vi "Refresh Scalar Channels.vi"(6 "scalar channels":T1[](array[typedef]) {"Data Type" format="%.0x"}, 8 "error in (no error)":errorcluster, 9 "scalar type GUID":string, 11 "scalar section ref in":T3 format="%.0x") -> (0 "error out":errorcluster, 3 "scalar section ref out":T3 format="%.0x")   [LabVIEW 2020, in "FPGA Addon System Explorer.lvlib"]
uses:
  FPGA Addon System Explorer.lvlib
  <vilib>/NI VeriStand/Custom Device API/Custom Device Item Ref.ctl
  Addon Shared/Types/Register Information.ctl
  Addon Shared/Types/FPGA Addon Data Type.ctl
  <vilib>/NI VeriStand/Custom Device Tools/Custom Device Utility Library/NI VeriStand - Search for Item by GUID.vi
  <vilib>/NI VeriStand/Custom Device Tools/Custom Device Utility Library/Custom Device Utility Library.lvlib
  <vilib>/NI VeriStand/Custom Device API/Custom Device API.lvlib
  Addon Shared/FPGA Addon Shared.lvlib
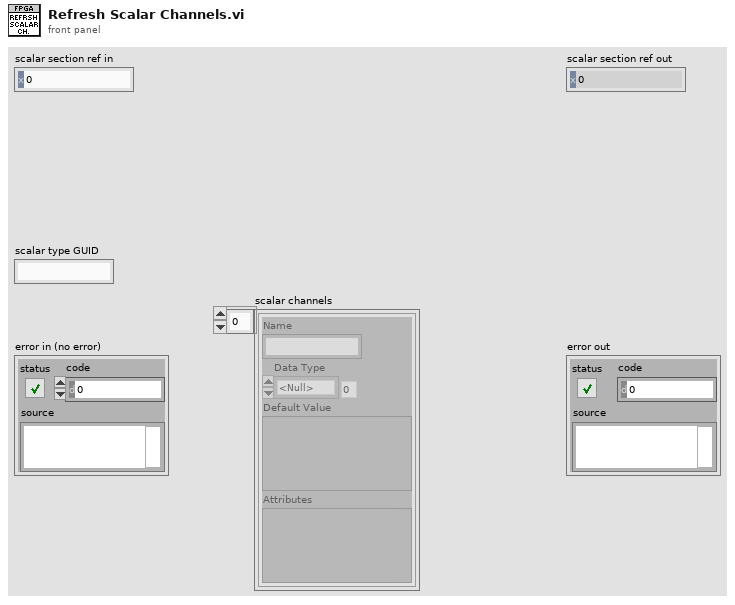
[diagram p1: front panel]
types:
  T1 = typedef "FPGA Addon Shared.lvlib/Register Information.ctl" = cluster{"Name":string, "Data Type":T2, "Default Value":variant, "Attributes":variant}
  T2 = typedef "FPGA Addon Shared.lvlib/FPGA Addon Data Type.ctl" = enum8{"<Null>", "I8", "I16", "I32", "I64", "U8", "U16", "U32", "U64", "SGL", "Boolean", "Analog PWM In Settings", "Analog PWM In", "Digital PWM In Settings", "Digital PWM In", "Digital PWM Out", "Sine Out", "FXP", "FXP+/-24.5", "FXP+/-16.5", "FXP+/-32.8", "FXP+/-64.32", "FXP+/-16.7", "FXP+/-20.5", "FXP+/-27.5", "FXP+/-32.16", "FXP+16.3", "FXP+18.3", "Digital Static In", "Digital Static Out", "Digital Static In Settings", "Digital WSS Out", "Quad Encoder Settings", "Quad Encoder In", "Group"}
  T3 = typedef "Custom Device API.lvlib/Custom Device Item Ref.ctl" = u64
  T4 = typedef "FPGA Addon System Explorer.lvlib/Output Scalar.ctl" = cluster{"Bitfile Name":string, "SysDef Channel Name":string, "Data Type":T2, "Default Value":variant, "Item Ref":T3}
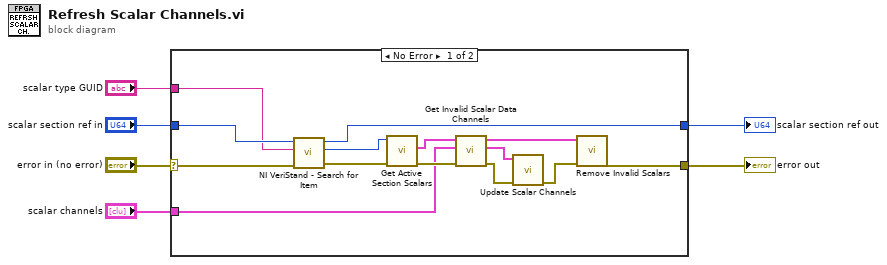
[diagram p0: block diagram]
diagram:
  n1 = case shown="No Error" "error in (no error)" {
    selector: "error in (no error)" -> [w8 w22]
    tunnel: "scalar section ref in" -> [w20 w21]
    tunnel: "scalar type GUID" -> [w19 _]
    tunnel: [w18 w21] -> w4
    tunnel: [w7 w22] -> w3
    tunnel: "scalar channels" -> [w13 _]
    frame No Error {
      n2 = call-poly <vilib>:"NI VeriStand - Search for Item.vi"("error in"=w8, "Item GUID"=w19, "Section Ref in"=w20) -> ("error out"=w16:errorcluster, "Item Ref"=w17:T3, "Section Ref out"=w18:T3)  [unwired: 5 in, 1 out]
      n3 = call "Get Active Section Scalars.vi"("error in"=w16, "section ref in"=w17) -> ("error out"=w15:errorcluster, "section scalars out"=w14:T4[])  [unwired: 7 in, 1 out]
      n4 = call "Get Invalid Scalar Data Channels.vi"("error in (no error)"=w15, "new bitfile scalar channels"=w13, "old bitfile scalar channels"=w14) -> ("error out"=w12:errorcluster, "valid scalar channels"=w10:T4[], "invalid scalar channels"=w9:T4[])  [unwired: 6 in]
      n5 = call "Update Scalar Channels.vi"("error in (no error)"=w12, "valid scalar channels"=w10) -> ("error out"=w11:errorcluster)  [unwired: 9 in]
      n6 = call "Remove Invalid Scalars.vi"("error in (no error)"=w11, "invalid scalar data channels"=w9) -> ("error out"=w7:errorcluster)  [unwired: 9 in]
    }
    frame Error {
    }
  }
  "scalar section ref out" <- w4
  "error out" <- w3
